vi "Constant_ADONetCore.vi"() -> (0 "ADOMapper NetCore":refnum<class "ADOMapper.lvclass">)   [LabVIEW 2026, in "ORM_API_NetCore.lvlib"]
uses:
  ORM_API_NetCore.lvlib
  <vilib>/Viviota/shared/ORM_ADONetCore.lvlibp/ADOMapper/ADOMapper.lvclass
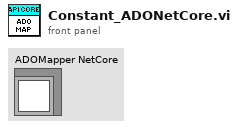
[diagram p1: front panel]
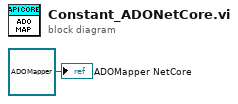
[diagram p0: block diagram]
diagram:
  "ADOMapper NetCore" <- refnum<class "ADOMapper.lvclass"> refnum ("ORM_ADONetCore.lvlibp:ADOMapper.lvclass")
